vi "PV_TimeSyncClient_Test.vi"() -> ()   [LabVIEW 2019]
uses:
  <vilib>/Rock Robotics/WPI/ThirdParty/PhotonVisionLib/PhotonVisionLib.lvlib
  <vilib>/Rock Robotics/WPI/ThirdParty/PhotonVisionLib/SubVI/PhotonVision_Globals.vi
panel:
  out "PV_TimeSyncClientLastSentSrcPort":u16
  out "PV_TimeSyncClientRcvSrcPort":u32
  out "PV_TimeSyncClientRcvIP":string
  out "PV_TimeSyncClientLoopCnt":i32
  in  "ServerIPAddress":string="127.0.0.1"
  out "PV_TimeSyncClientLastRcvTime":i64
  out "PV_TimeSyncClientLastRcvVer":i8
  out "PV_TimeSyncClientLastSentTime":i64
  out "PV_TimeSyncClientReadErr":bool
  out "PV_TimeSyncClientStop":bool
  out "PV_TimeSyncClientTimeOffset":i64
  out "PV_TimeSyncClientWriteErr":bool
  out "PV_TimeSyncClientLastRcvId":i8
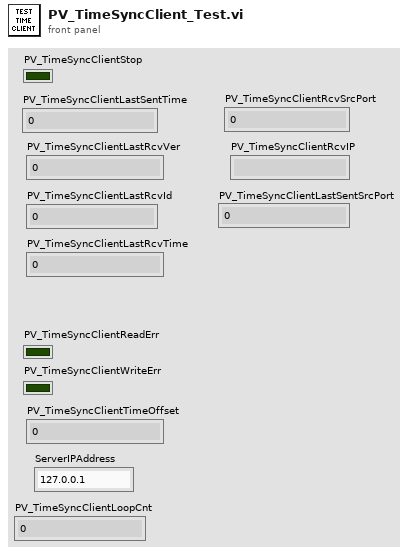
[diagram p1: front panel]
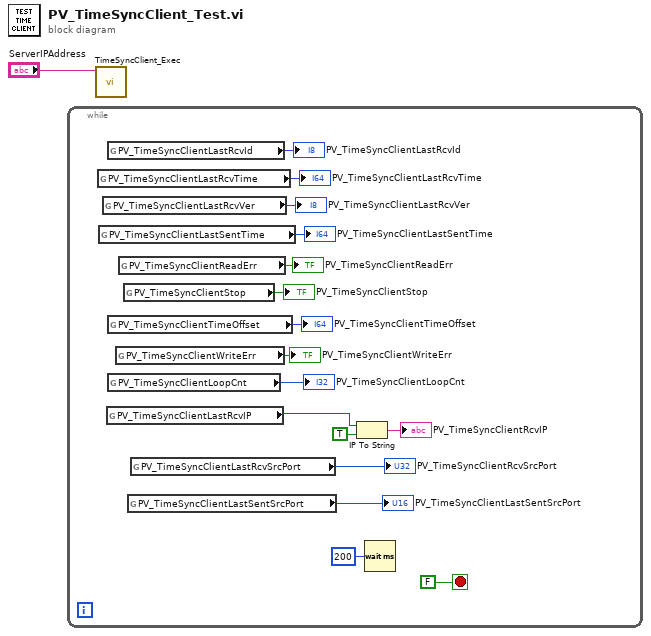
[diagram p0: block diagram]
diagram:
  n1 = while {
    stop <- FALSE stop-if-true
    n2 = global read "PhotonVision_Globals.vi" "PV_TimeSyncClientLastRcvTime"() -> (→"PV_TimeSyncClientLastRcvTime":i64)
    n3 = global read "PhotonVision_Globals.vi" "PV_TimeSyncClientLastSentTime"() -> (→"PV_TimeSyncClientLastSentTime":i64)
    n4 = global read "PhotonVision_Globals.vi" "PV_TimeSyncClientLastRcvVer"() -> (→"PV_TimeSyncClientLastRcvVer":i8)
    n5 = global read "PhotonVision_Globals.vi" "PV_TimeSyncClientLastRcvIP"() -> (w3:u32)
    n6 = global read "PhotonVision_Globals.vi" "PV_TimeSyncClientLastRcvId"() -> (→"PV_TimeSyncClientLastRcvId":i8)
    n7 = global read "PhotonVision_Globals.vi" "PV_TimeSyncClientTimeOffset"() -> (→"PV_TimeSyncClientTimeOffset":i64)
    n8 = global read "PhotonVision_Globals.vi" "PV_TimeSyncClientLoopCnt"() -> (→"PV_TimeSyncClientLoopCnt":i32)
    n9 = global read "PhotonVision_Globals.vi" "PV_TimeSyncClientWriteErr"() -> (→"PV_TimeSyncClientWriteErr":bool)
    n10 = global read "PhotonVision_Globals.vi" "PV_TimeSyncClientReadErr"() -> (→"PV_TimeSyncClientReadErr":bool)
    n11 = global read "PhotonVision_Globals.vi" "PV_TimeSyncClientStop"() -> (→"PV_TimeSyncClientStop":bool)
    n12 = global read "PhotonVision_Globals.vi" "PV_TimeSyncClientLastSentSrcPort"() -> (→"PV_TimeSyncClientLastSentSrcPort":u16)
    n13 = global read "PhotonVision_Globals.vi" "PV_TimeSyncClientLastRcvSrcPort"() -> (→"PV_TimeSyncClientRcvSrcPort":u16)
    n14 = IP To String(1:TRUE ("dot notation? (F)"), 2:w3) -> (0:→"PV_TimeSyncClientRcvIP":string)
    n15 = Wait (ms)(milliseconds to wait=u32 200) -> ()  [unwired: 1 out]
  }
  n16 = call <vilib>:"TimeSyncClient_Exec.vi"("ServerIPAddress"="ServerIPAddress") -> ()  [unwired: 11 in]
